vi "TCP Server Engine.vi"(8 "error in (no error)":errorcluster, 9 "User Events":T1, 10 "Port (0)":i32, 11 "Service Name":string) -> (0 "error out":errorcluster)   [LabVIEW 2016, in "SLL Easy API via TCP.lvclass"]
uses:
  SLL Easy API via TCP.lvclass
  _Typedefs/User Events to TCP Engine.ctl
  _Typedefs/TCP Event Data.ctl
  <vilib>/Utility/error.llb/DialogType.ctl
  SLL Queued State Machine/Queue Driver/Create Queue.vi
  SLL Queued State Machine/Queue Driver/Enqueue an Item to Queue.vi
  SLL Queued State Machine/Queue Driver/Dequeue Queue.vi
  SLL Queued State Machine/Queue Driver/Enqueue N Items.vi
  SLL Queued State Machine/Queue Driver/Flush Queue.vi
  SLL Queued State Machine/Queue Driver/Release Queue.vi
  SLL Queued State Machine/SLL QSM.lvlib
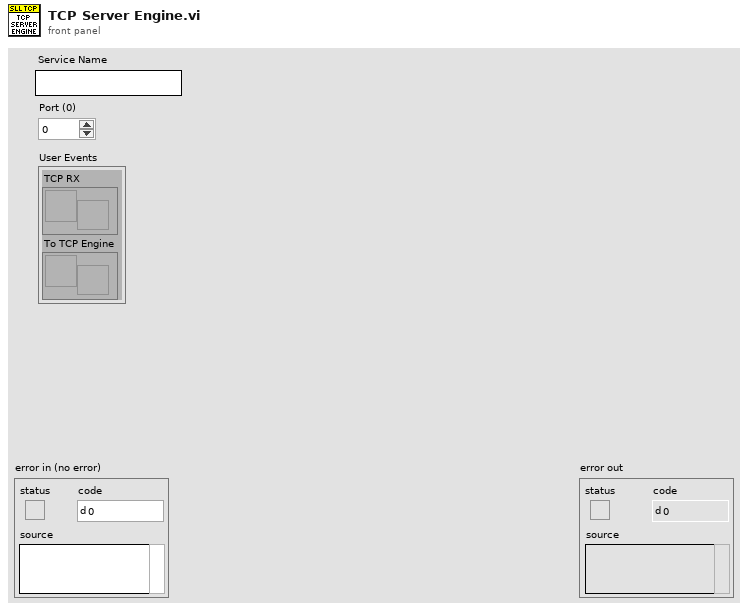
[diagram p1: front panel]
types:
  T1 = typedef "SLL Easy API via TCP.lvclass/User Events to TCP Engine.ctl" = cluster{"TCP RX":refnum<user-event>, "To TCP Engine":refnum<user-event>}
  T2 = cluster{"Flags":cluster{"Source Code?":bool}, "Listener ID":refnum<k5>, "Connection ID[]":refnum<k5>[], "User Events":T1}
  T3 = typedef "DialogType.ctl" = u16
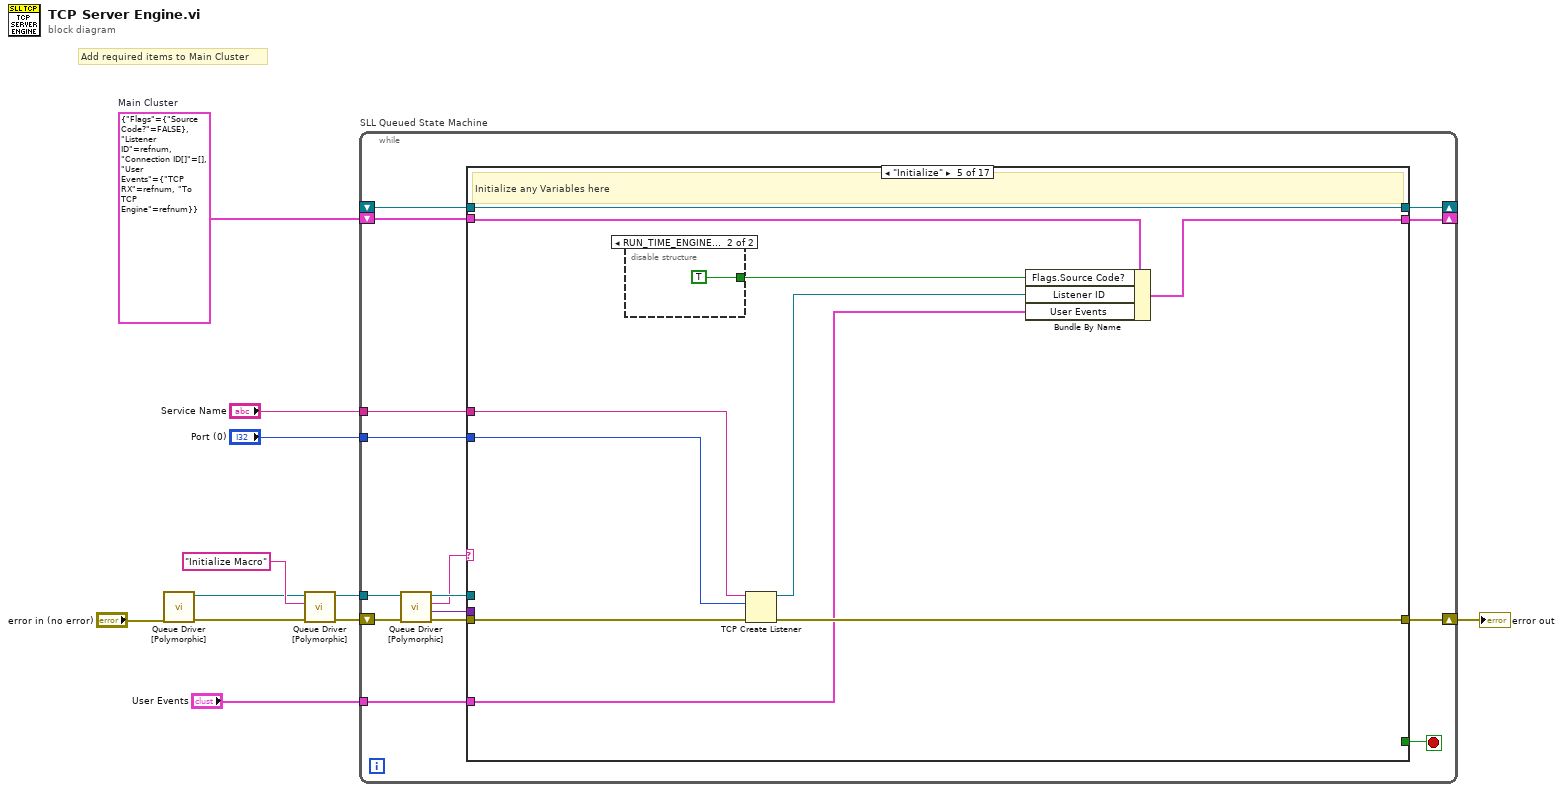
[diagram p0: block diagram]
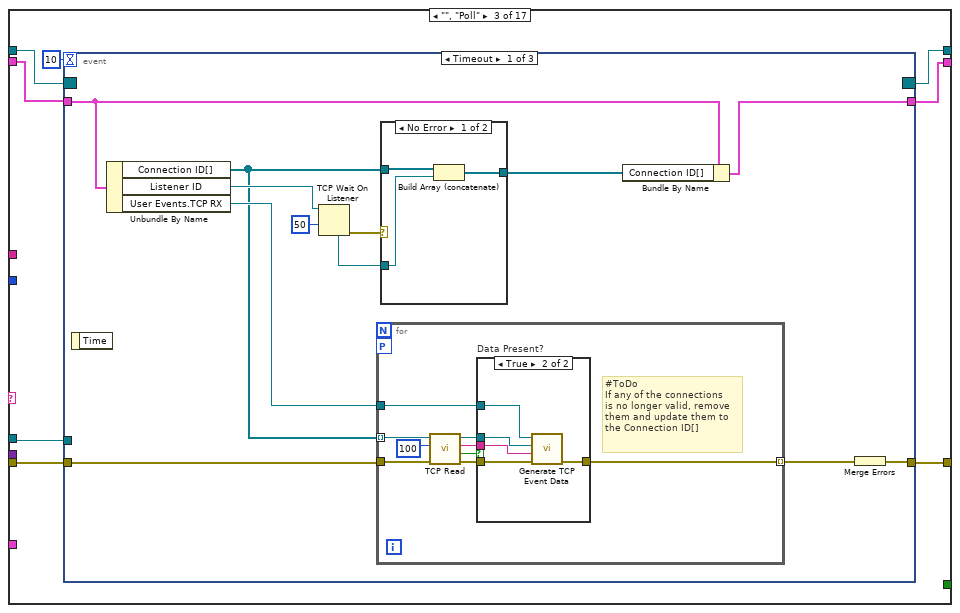
[diagram p4: hidden frame]
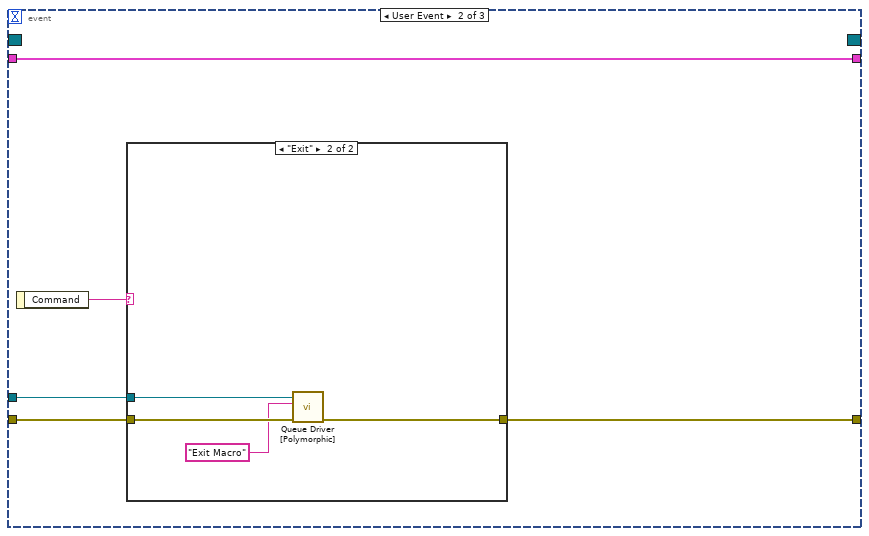
[diagram p7: hidden frame]
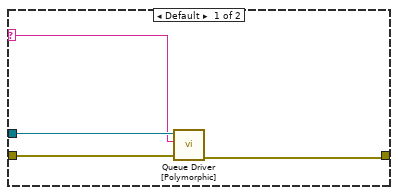
[diagram p8: hidden frame]
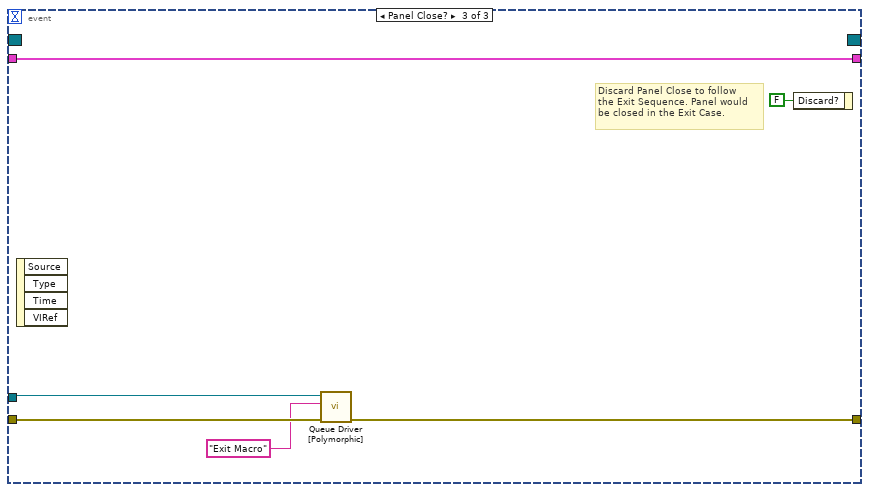
[diagram p9: hidden frame]
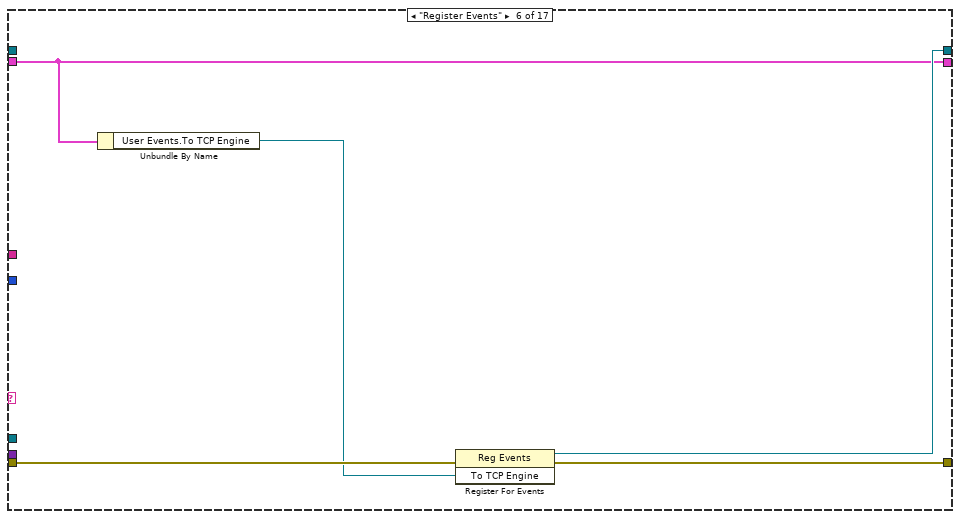
[diagram p12: hidden frame]
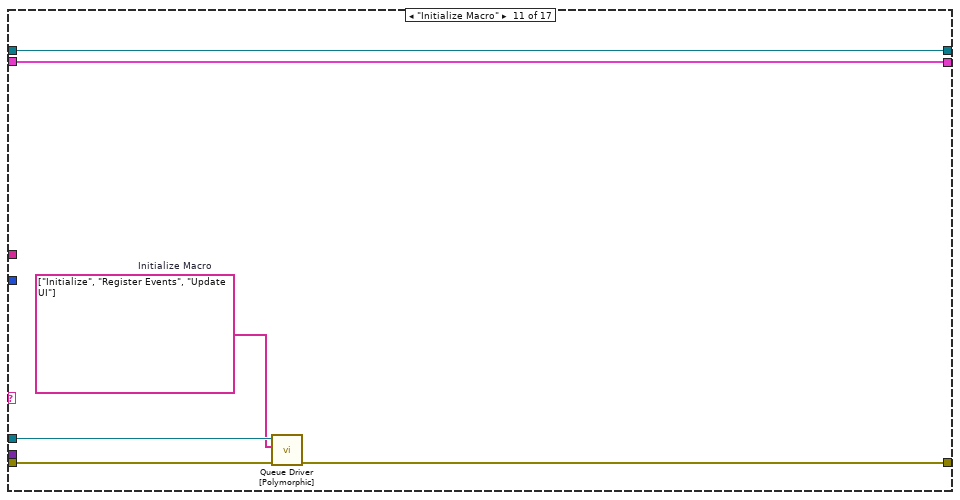
[diagram p17: hidden frame]
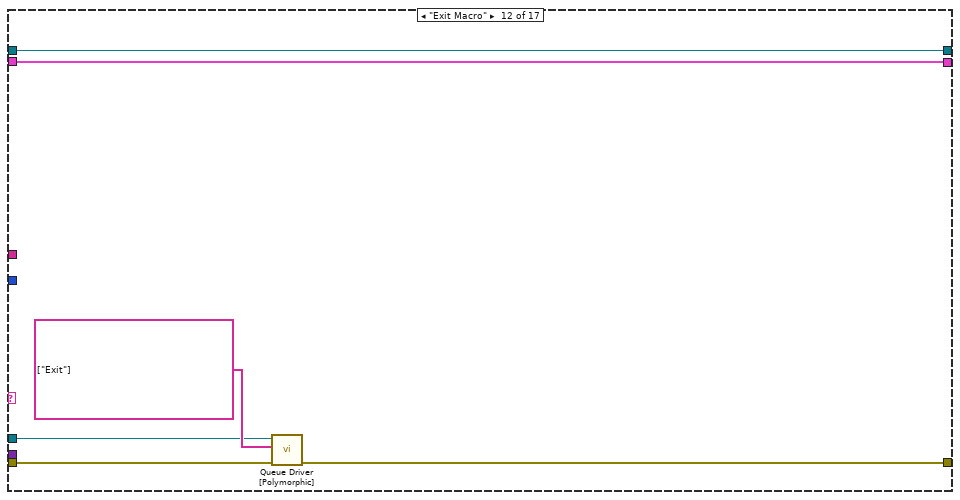
[diagram p18: hidden frame]
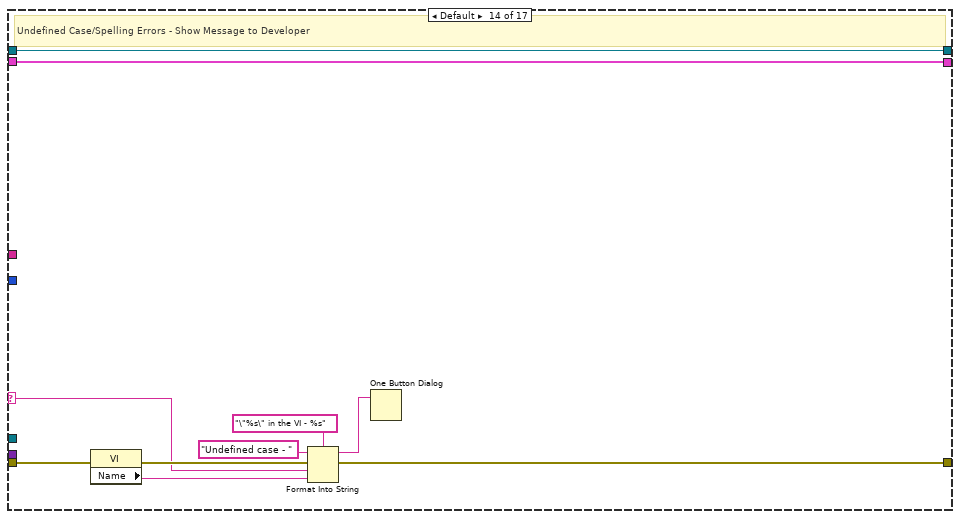
[diagram p20: hidden frame]
diagram:
  w11 = T2 {"Flags"={"Source Code?"=FALSE}, "Listener ID"=refnum, "Connection ID[]"=[], "User Events"={"TCP RX"=refnum, "To TCP Engine"=refnum}}  # Main Cluster
  # "Add required items to Main Cluster"
  n1 = call-poly "Queue Driver [Polymorphic].vi"("Error In"="error in (no error)") -> ("Error Out"=w9:errorcluster, "Queue Ref"=w5:refnum<queue>)  [unwired: 9 in]
  n2 = call-poly "Queue Driver [Polymorphic].vi"("Error In"=w9, "Item to Add"="Initialize Macro", "Queue Ref In"=w5) -> ("Error Out"=w10:errorcluster, "Queue Ref Out"=w4:refnum<queue>)  [unwired: 7 in]
  n3 = while "SLL Queued State Machine" {
    shift-right: [w24] -> w7
    shift-left: w10 -> [w26]
    shift-right: [w21] -> _
    shift-left: _ -> [w20]
    shift-right: [w19] -> _
    shift-left: w11 -> [w18]
    tunnel: w4 -> [w16]
    tunnel: "Service Name" -> [w14]
    tunnel: "Port (0)" -> [w13]
    tunnel: "User Events" -> [w12]
    stop <- w23 stop-if-true
    n4 = call-poly "Queue Driver [Polymorphic].vi"("Error In"=w26, "Queue Ref In"=w16) -> ("Error Out"=w25:errorcluster, "Data"=w15:variant, "Dequeue"=w17:string, "Queue Ref Out"=w22:refnum<queue>)  [unwired: 6 in]
    n5 = case "QSM Case Structure" shown="\"Initialize\"" w17 {
      selector: w17 -> [_ _ _ _ _ _ _ _ _ _ _ _ _ w137 _ _ _]
      tunnel: w25 -> [w29 w32 w38 w93 w99 w109 w112 w115 w118 w121 w125 w131 w136 w140 w152 w155 w168]
      tunnel: [w29 w32 w39 w93 w98 w108 w112 w115 w118 w121 w124 w130 w136 w143 w150 w155 w164] -> w24
      tunnel: [_ _ _ _ _ _ _ _ _ _ _ _ _ _ _ _ TRUE] -> w23
      tunnel: [w28 w31 w37 w92 w103 w107 w111 w114 w117 w120 w127 w133 w135 w146 w149 w154 w167] -> w21
      tunnel: w20 -> [w28 w31 w36 w92 w103 _ w111 w114 w117 w120 w127 w133 w135 w146 w149 w154 w167]
      tunnel: [w27 w30 w34 w91 w100 w106 w110 w113 w116 w119 w126 w132 w134 w145 w148 w153 w166] -> w19
      tunnel: w18 -> [w27 w30 w35 w91 w101 w106 w110 w113 w116 w119 w126 w132 w134 w145 w148 w153 w166]
      tunnel: w22 -> [_ _ w33 _ _ _ _ _ _ _ w123 w128 _ _ _ _ w157]
      tunnel: w15 -> [_ _ _ _ _ _ _ _ _ _ _ _ _ _ _ _ _]
      tunnel: w14 -> [_ _ _ _ w96 _ _ _ _ _ _ _ _ _ _ _ _]
      tunnel: w13 -> [_ _ _ _ w95 _ _ _ _ _ _ _ _ _ _ _ _]
      tunnel: w12 -> [_ _ _ _ w94 _ _ _ _ _ _ _ _ _ _ _ _]
      frame "/*** Read Me ***/" {
        # "General Purpose Queue Based State Machine for Any Use Case (main application, module, pop up message etc)\n\nAdvantages:\n1. No Need to Pass Queue References between Queue Driver VIs.\n2. This template can be safely used in multiple parallel running modules without any issues.\n3. This template can also be safely used even in cases where the VI is configured to be a Clone, where multiple \ninstances of the VI could be executing concurrently.\n\nHow to Use:\n1. Add necessary items to the Main Cluster.\n2. Use the Polymorphic Queue Driver for doing any queue operations. There is no need to pass the queue driver\nreference, as the Queue Driver automatically infers the reference based on the VI instance from which it is called.\n3. Add any required user events in the \"Register Events\" case. Ignore if not needed.\n4. Use \"Sequences\" section for defining any list of state calls, which could be used in multiple places. \nEg: Initialize Sequence, might be needed if we need to any reinitialization."
      }
      frame "/**** Poll ****/" {
      }
      frame "", "Poll" {
        n6 = event shown="[0] Timeout" {
          selector: w36 -> [_ _ _]
          dyn-events: [_ _ _] -> w37
          timeout: 10 -> [_ _ _]
          tunnel: [w43 w74 w89] -> w39
          tunnel: w38 -> [w45 w75 w90]
          tunnel: w35 -> [w48 w76 w88]
          tunnel: [w47 w76 w88] -> w34
          tunnel: w33 -> [_ w72 w86]
          event Timeout {
            n7 = event-data() -> ()  [unwired: 1 in, 1 out]
            n8 = Unbundle By Name(w48) -> ("Connection ID[]"=w41:refnum<k5>[], "Listener ID"=w52:refnum<k5>, "User Events.TCP RX"=w42:refnum<user-event>)
            n9 = TCP Wait On Listener(9:50 ("timeout ms (wait forever: -1)"), 11:w52) -> (0:w50:errorcluster, 4:w49:refnum<k5>)  [unwired: 2 in, 3 out]
            n10 = for {
              tunnel: w41 -> [w61] mode=indexing
              workers-P: _ -> [_]
              tunnel: w45 -> [w60]
              tunnel: [w58] -> w44 mode=indexing
              tunnel: w42 -> [w54]
              # "#ToDo\nIf any of the connections\nis no longer valid, remove\nthem and update them to\nthe Connection ID[]"
              n11 = call "TCP Read.vi"("error in (no error)"=w60, "timeout ms (1000)"=100, "Connection ID In"=w61) -> ("error out"=w59:errorcluster, "Data Available?"=w56:bool, "Read Data"=w57:string, "Connection ID Out"=w55:refnum<k5>)  [unwired: 5 in]
              n12 = case "Data Present?" shown="True" w56 {
                tunnel: w59 -> [w62 w67]
                tunnel: [w62 w66] -> w58
                tunnel: w57 -> [_ w63]
                tunnel: w54 -> [_ w65]
                tunnel: w55 -> [_ w64]
                frame False {
                }
                frame True {
                  n13 = call "Generate TCP Event Data.vi"("error in (no error)"=w67, "TCP Data"=w63, "Connection ID"=w64, "User Events.TCP RX"=w65) -> ("error out"=w66:errorcluster)  [unwired: 7 in]
                }
              }
            }
            n14 = case shown="No Error" w50 {
              tunnel: w41 -> [w70 w71]
              tunnel: w49 -> [w69 _]
              tunnel: [w68 w71] -> w46
              frame No Error {
                n15 = Build Array (concatenate)(w70, w69) -> (w68:refnum<k5>[])
              }
              frame Error {
              }
            }
            n16 = Bundle By Name(cluster=w48, "Connection ID[]"=w46) -> (w47:T2)
            n17 = Merge Errors(w44) -> (w43:errorcluster)
          }
          event User Event {
            n18 = event-data() -> ("Command"=w73:string)  [unwired: 1 in]
            n19 = case shown="\"Exit\"" w73 {
              selector: w73 -> [w77 _]
              tunnel: w75 -> [w80 w84]
              tunnel: [w79 w83] -> w74
              tunnel: w72 -> [w78 w82]
              frame Default {
                n20 = call-poly "Queue Driver [Polymorphic].vi"("Error In"=w80, "Item to Add"=w77, "Queue Ref In"=w78) -> ("Error Out"=w79:errorcluster)  [unwired: 7 in, 1 out]
              }
              frame "Exit" {
                n21 = call-poly "Queue Driver [Polymorphic].vi"("Error In"=w84, "Item to Add"="Exit Macro", "Queue Ref In"=w82) -> ("Error Out"=w83:errorcluster)  [unwired: 7 in, 1 out]
              }
            }
          }
          event Panel Close? {
            # "Discard Panel Close to follow\nthe Exit Sequence. Panel would\nbe closed in the Exit Case."
            n22 = event-data() -> ()  [unwired: 1 in, 4 out]
            n23 = call-poly "Queue Driver [Polymorphic].vi"("Error In"=w90, "Item to Add"="Exit Macro" ("Enqueue"), "Queue Ref In"=w86) -> ("Error Out"=w89:errorcluster)  [unwired: 7 in, 1 out]
            n24 = event-data ("Event Filter Node")("Discard?"=FALSE) -> ()  [unwired: 1 in, 1 out]
          }
        }
      }
      frame "/**** Initialize ****/" {
      }
      frame "Initialize" {
        # "Initialize any Variables here"
        n25 = disable-structure "Conditional Disable Structure" shown="RUN_TIME_ENGINE==False" {
          disable-tunnel: [_ TRUE] -> w102
          frame condition #0 {
          }
          frame condition #1 (active) {
          }
        }
        n26 = TCP Create Listener(8:w99, 10:w95, 11:w96) -> (0:w98:errorcluster, 3:w97:refnum<k5>)  [unwired: 2 in, 1 out]
        n27 = Bundle By Name(cluster=w101, "Flags.Source Code?"=w102, "Listener ID"=w97, "User Events"=w94) -> (w100:T2)
      }
      frame "Register Events" {
        n28 = Unbundle By Name(w106) -> ("User Events.To TCP Engine"=w105:refnum<user-event>)
        n29 = register-events(error in=w109, w105) -> (reference out=w107:refnum<event-registration>, error out=w108:errorcluster)  [unwired: 1 in]
      }
      frame "/*** Custom Case Splitter ***/" {
      }
      frame "/*** User Interface Actions ***/" {
        # "Duplicate this case to create additional case splitters for readability"
      }
      frame "Update UI" {
        # "Update Front Panel Controls in this Case"
      }
      frame "/*** Macros ***/" {
      }
      frame "Initialize Macro" {
        w122 = string[] ["Initialize", "Register Events", "Update UI"]  # Initialize Macro
        n30 = call-poly "Queue Driver [Polymorphic].vi"("Error In"=w125, "Enqueue N"=w122, "Queue Ref In"=w123) -> ("Error Out"=w124:errorcluster)  [unwired: 7 in, 1 out]
      }
      frame "Exit Macro" {
        n31 = call-poly "Queue Driver [Polymorphic].vi"("Error In"=w131, "Enqueue N"=string[] ["Exit"], "Queue Ref In"=w128) -> ("Error Out"=w130:errorcluster)  [unwired: 7 in, 1 out]
      }
      frame "/*** Error Handler ***/" {
      }
      frame Default {
        # "Undefined Case/Spelling Errors - Show Message to Developer"
        n32 = property on="Property Node" class="VI"(error in=w140) -> (error out=w139:errorcluster, "Name"=w138:string)  [unwired: 1 in, 1 out]
        n33 = Format Into String(format string="\"%s\" in the VI - %s" ("message"), initial string="Undefined case - ", error in=w139, w137, w138) -> (resulting string=w141:string, error out=w143:errorcluster)
        n34 = One Button Dialog(message=w141) -> ()  [unwired: 1 in, 1 out]
      }
      frame "Error" {
        w147 = T3 2 items=["no dialog", "OK message", "continue or stop message", "OK message + warnings", "continue/stop + warnings"] ("type of dialog (OK msg:1)")
        # "Handle the Error"
        n35 = call <vilib>:"Simple Error Handler.vi"("type of dialog (OK msg:1)"=w147, "error in (no error)"=w152) -> ("error out"=w151:errorcluster)  [unwired: 3 in, 4 out]
        n36 = call <vilib>:"Clear Errors.vi"("error in (no error)"=w151) -> ("error out"=w150:errorcluster)  [unwired: 5 in, 1 out]
      }
      frame "/**** Exit ****/" {
      }
      frame "Exit" {
        n37 = call-poly "Queue Driver [Polymorphic].vi"("Error In"=w168, "Queue Ref In"=w157) -> ("Error Out"=w169:errorcluster, "Queue Ref Out"=w156:refnum<queue>)  [unwired: 7 in, 1 out]
        n38 = Unbundle By Name(w166) -> ("Flags.Source Code?"=w159:bool)
        n39 = call-poly "Queue Driver [Polymorphic].vi"("Error In"=w169, "Queue Ref In"=w156) -> ("Error Out"=w165:errorcluster)  [unwired: 9 in]
        n40 = Call Chain() -> (call chain=w163:string[])
        n41 = Array Size(array=w163) -> (size(s)=w162:i32)
        n42 = Equal?(x=w162, y=1) -> (x = y?=w160:bool)
        n43 = And(x=w159, y=w160) -> (x .and. y?=w158:bool)
        n44 = case "Skip Panel Close when in Source\nCode and is the top most caller" shown="True" w158 {
          tunnel: w165 -> [w172 w174]
          tunnel: [w173 w174] -> w164
          frame False {
            # "Close Panel"
            n45 = invoke on="Invoke Node" class="VI" method="FP.Close"() -> (error out=w171:errorcluster)  [unwired: 3 in, 2 out]
            n46 = Merge Errors(w172, w171) -> (w173:errorcluster)
          }
          frame True {
            # "Do Not Close Panel"
          }
        }
      }
    }
  }
  "error out" <- w7
